vi "Stream to Image Files-example-v2.vi"() -> ()   [LabVIEW 2025]
doc: "The Stream to Image Files example shows how to save images to PNG files in parallel when using a grab acquisition. Images acquired from a camera are stored in a manager and each worker loop removes an image from the manager to save to disk. When the save to disk is complete, the image is added back to the manager so it can be used to copy acquired images into again. It is recommended to use the Stream to Image Files (Optimized Performance) example if your camera settings work with a ring acquisition."
uses:
  VIs_needed/Grab Manager Mode.ctl
  <vilib>/vision/driver/IMAQdx.llb/IMAQdx Buffer Number Mode.ctl
  <vilib>/Utility/High Resolution Relative Seconds.vi
  <vilib>/vision/driver/NI_Vision_Acquisition_Software.lvlib
  <resource>/objmgr/imaqdx.rc
panel:
  out "Images Acquired Per Second":dbl
  in  "Skip Count":u32
  out "Images Behind":i32
  out "Images Saved Per Second":dbl
  in  "Number of Images":u32=30
  out "Destination Folder":path
  out "Write Speed":dbl(graph) caption="Image File Write Speed"
  in  "Camera Name":refnum<k21> caption="IMAQdx Session"
  in  "Stop":bool
  # "Overview: Demonstrates how to stream images to disk in parallel when using a ring acquisition.\nRequirements: Vision Acquisition Software\nInstructions:\n1. Select the Camera Name\n2. Run the VI\n3. Reduce the Number of Workers to see if the streaming of images can keep up with fewer workers.\n4. Increase the Skip Count if Images Behind is greater than 0."
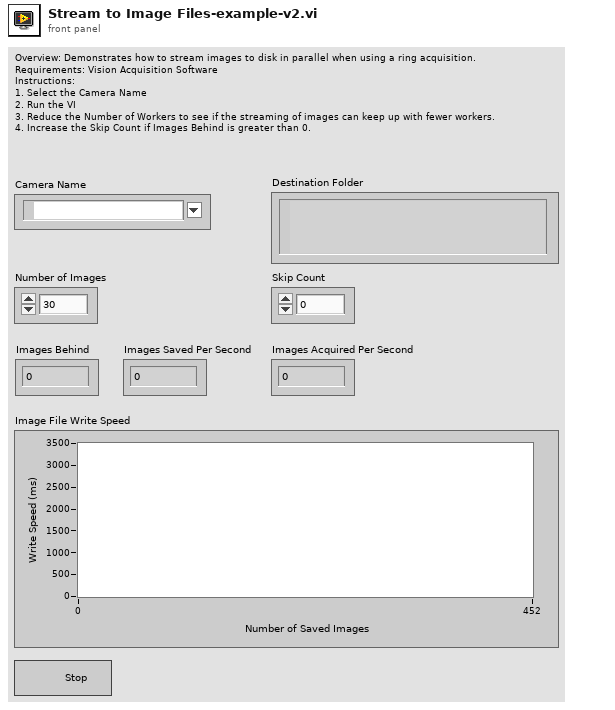
[diagram p1: front panel]
types:
  T1 = cluster{"Number of Processing Images":u32, "Image Border Size":u32}
  T2 = typedef "Grab Manager Mode.ctl" = enum16{"Create Processing Images", "Lock", "Add Acquired Image", "Get Acquired Image", "Unlock", "Dispose Processing Images"}
  T3 = typedef "IMAQdx.ctl" = refnum<k21>
  T4 = typedef "NI_Vision_Acquisition_Software.lvlib/IMAQdx Buffer Number Mode.ctl" = enum32{"Next", "Last", "Buffer Number", "Every", "Last New"}
  T5 = typedef "IMAQ Image.ctl" = refnum<image>
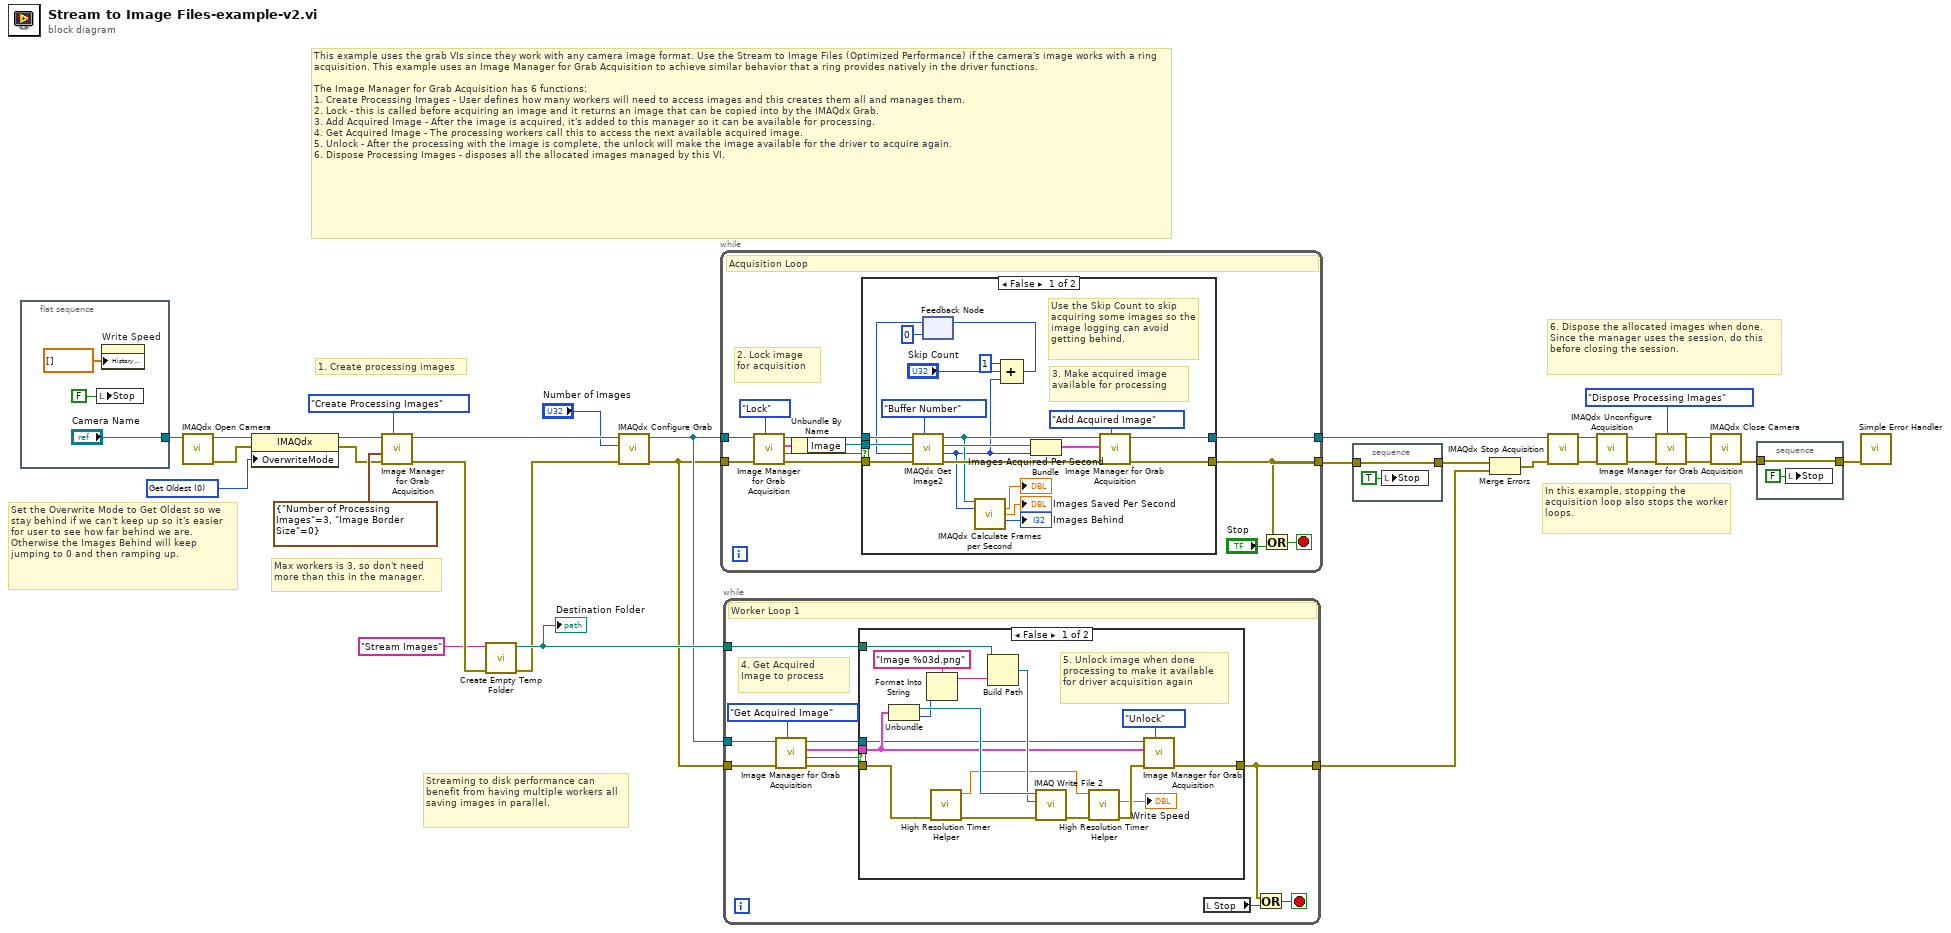
[diagram p0: block diagram]
diagram:
  w19 = u32 0 items=["Get Oldest"=0, "Fail"=2, "Get Newest"=3] ("OverwriteMode")
  # "6. Dispose the allocated images when done. Since the manager uses the session, do this before closing the session."
  # "1. Create processing images"
  # "This example uses the grab VIs since they work with any camera image format. Use the Stream to Image Files (Optimized Performance) if the camera's image works with a ring acquisition. This example uses an Image Manager for Grab Acquisition to achieve similar behavior that a ring provides natively in the driver functions.\n\nThe Image Manager for Grab Acquisition has 6 functions:\n1. Create Processing Images - User defines how many workers will need to access images and this creates them all and manages them.\n2. Lock - this is called before acquiring an image and it returns an image that can be copied into by the IMAQdx Grab.\n3. Add Acquired Image - After the image is acquired, it's added to this manager so it can be available for processing.\n4. Get Acquired Image - The processing workers call this to access the next available acquired image.\n5. Unlock - After the processing with the image is complete, the unlock will make the image available for the driver to acquire again.\n6. Dispose Processing Images - disposes all the allocated images managed by this VI."
  # "Set the Overwrite Mode to Get Oldest so we stay behind if we can't keep up so it's easier for user to see how far behind we are. Otherwise the Images Behind will keep jumping to 0 and then ramping up."
  # "Max workers is 3, so don't need more than this in the manager."
  # "In this example, stopping the acquisition loop also stops the worker loops."
  # "Streaming to disk performance can benefit from having multiple workers all saving images in parallel."
  n1 = flat-sequence {
    tunnel: ["Camera Name"] -> w30
    frame #0 {
      n2 = local write "Stop"(FALSE ("Stop")) -> ()
      n3 = property on="Write Speed" class="WFChart (strict)"("History Data"=dbl[] []) -> ()  [unwired: 2 in, 2 out]
    }
  }
  n4 = call <vilib>:"IMAQdx Open Camera.vi"("Session In"=w30) -> ("error out"=w10:errorcluster, "Session Out"=w20:T3)  [unwired: 2 in, 7 out]
  n5 = property class="IMAQdx"(reference=w20, error in=w10, "OverwriteMode"=w19) -> (reference out=w9:T3, error out=w8:errorcluster)
  n6 = call "Image Manager for Grab Acquisition.vi"("Mode"=Grab_Manager_Mode."Create Processing Images", "error in (no error)"=w8, "Init Settings"=T1 {"Number of Processing Images"=3, "Image Border Size"=0}, "Session In"=w9) -> ("error out"=w7:errorcluster, "Session Out"=w5:T3)  [unwired: 4 in, 2 out]
  n7 = call "Create Empty Temp Folder.vi"("error in (no error)"=w7, "Folder Name"="Stream Images") -> ("error out"=w4:errorcluster, "Empty Temp Folder"=w21:path)  [unwired: 8 in]
  "Destination Folder" <- w21
  n8 = call <vilib>:"IMAQdx Configure Grab.vi"("error in"=w4, "Number of Buffers"="Number of Images", "Session In"=w5) -> ("error out"=w2:errorcluster, "Session Out"=w3:T3)  [unwired: 7 in]
  n9 = while {
    tunnel: w2 -> [w43]
    tunnel: w3 -> [w40]
    tunnel: [w41] -> w26
    tunnel: [w42] -> w25
    stop <- w44 stop-if-true
    # "2. Lock image for acquisition"
    # "Acquisition Loop"
    n10 = call "Image Manager for Grab Acquisition.vi"("Mode"=Grab_Manager_Mode."Lock", "error in (no error)"=w43, "Session In"=w40) -> ("error out"=w36:errorcluster, "No Available Image"=w37:bool, "Image Settings Out"=w35:cluster{"Image":T5, "Buffer Number":u32}, "Session Out"=w38:T3)  [unwired: 5 in]
    n11 = Unbundle By Name(w35) -> ("Image"=w34:T5)
    n12 = case shown="False" w37 {
      tunnel: [w57 w67] -> w41
      tunnel: [w56 w66] -> w42
      tunnel: w38 -> [w65 w67]
      tunnel: w36 -> [w64 w66]
      tunnel: w34 -> [w58 _]
      frame False {
        # "3. Make acquired image available for processing"
        # "Use the Skip Count to skip acquiring some images so the image logging can avoid getting behind."
        n13 = feedback #1(u32 0) -> (w47:u32)
        n14 = call <vilib>:"IMAQdx Get Image2.vi"("Buffer Number Mode (Next)"=IMAQdx_Buffer_Number_Mode."Buffer Number", "error in"=w64, "Buffer Number In"=w47, "Image In"=w58, "Session In"=w65) -> ("error out"=w60:errorcluster, "Buffer Number Out"=w51:u32, "Image Out"=w62:T5, "Session Out"=w55:T3)  [unwired: 3 in]
        n15 = call <vilib>:"IMAQdx Calculate Frames per Second.vi"("Session In"=w55, "Buffer Number"=w51) -> ("Acquired Frames per Second"=→"Images Acquired Per Second":dbl, "Processed Frames per Second"=→"Images Saved Per Second":dbl, "Images Behind"=→"Images Behind":i32)  [unwired: 7 in, 4 out]
        n16 = Compound Arithmetic op=ADD(u32 1 ("value"), "Skip Count", w51) -> (w48:u32)
        n17 = feedback-in #1(w48) -> ()
        n18 = Bundle("Image Out"=w62, "Buffer Number Out"=w51) -> (w61:cluster{"Image Out":T5, "Buffer Number Out":u32})  [unwired: 1 in]
        n19 = call "Image Manager for Grab Acquisition.vi"("Mode"=Grab_Manager_Mode."Add Acquired Image", "error in (no error)"=w60, "Image Settings In"=w61, "Session In"=w55) -> ("error out"=w56:errorcluster, "Session Out"=w57:T3)  [unwired: 4 in, 2 out]
      }
      frame True {
        # "The Lock function already has a delay inside when no images are available to prevent loop from going too fast and starving the worker threads from getting processing time."
        # "Write to disk operation is taking longer so images aren't added back to manager. Wait until there is an available image"
      }
    }
    n20 = Or(x=w42, y="Stop") -> (x .or. y?=w44:bool)
  }
  n21 = while {
    tunnel: w2 -> [w74]
    tunnel: w21 -> [w76]
    tunnel: [w75] -> w22
    tunnel: w3 -> [w69]
    stop <- w78 stop-if-true
    # "4. Get Acquired Image to process"
    # "Worker Loop 1"
    n22 = call "Image Manager for Grab Acquisition.vi"("Mode"=Grab_Manager_Mode."Get Acquired Image", "error in (no error)"=w74, "Session In"=w69) -> ("error out"=w70:errorcluster, "No Available Image"=w72:bool, "Image Settings Out"=w71:cluster{"Image":T5, "Buffer Number":u32}, "Session Out"=w68:T3)  [unwired: 5 in]
    n23 = case shown="False" w72 {
      tunnel: w70 -> [w84 w95]
      tunnel: w71 -> [w86 _]
      tunnel: [w88 w95] -> w75
      tunnel: w76 -> [w93 _]
      tunnel: w68 -> [w85 _]
      frame False {
        # "5. Unlock image when done processing to make it available for driver acquisition again"
        n24 = Unbundle(w86) -> ("Image"=w94:T5, "Buffer Number"=w90:u32)
        n25 = Format Into String(format string="Image %03d.png", w90) -> (resulting string=w92:string)  [unwired: 2 in, 1 out]
        n26 = call "High Resolution Timer Helper.vi"("error in (no error)"=w84) -> ("error out"=w83:errorcluster, "Current Time"=w80:dbl)  [unwired: 8 in, 1 out]
        n27 = Build Path(base path=w93, name or relative path=w92) -> (appended path=w89:path)
        n28 = call-poly "IMAQ Write File 2"("error in (no error)"=w83, "File Path"=w89, "Image"=w94) -> ("error out"=w82:errorcluster)  [unwired: 7 in, 1 out]
        n29 = call "High Resolution Timer Helper.vi"("error in (no error)"=w82, "Previous Time"=w80) -> ("error out"=w81:errorcluster, "Time Difference (ms)"=→"Write Speed":dbl)  [unwired: 7 in, 1 out]
        n30 = call "Image Manager for Grab Acquisition.vi"("Mode"=Grab_Manager_Mode."Unlock", "error in (no error)"=w81, "Image Settings In"=w86, "Session In"=w85) -> ("error out"=w88:errorcluster)  [unwired: 4 in, 3 out]
      }
      frame True {
        # "No acquired images to process"
      }
    }
    n31 = local read "Stop"() -> (w77:bool)
    n32 = Or(x=w75, y=w77) -> (x .or. y?=w78:bool)
  }
  n33 = stacked-sequence {
    tunnel: [w96] -> w24
    tunnel: w25 -> [w96]
    frame #0 {
      n34 = local write "Stop"(TRUE ("Stop")) -> ()
    }
  }
  n35 = Merge Errors(w24, w22) -> (w27:errorcluster)
  n36 = call <vilib>:"IMAQdx Stop Acquisition.vi"("error in"=w27, "Session In"=w26) -> ("error out"=w28:errorcluster, "Session Out"=w29:T3)  [unwired: 8 out]
  n37 = call <vilib>:"IMAQdx Unconfigure Acquisition.vi"("error in"=w28, "Session In"=w29) -> ("error out"=w17:errorcluster, "Session Out"=w18:T3)  [unwired: 8 out]
  n38 = call "Image Manager for Grab Acquisition.vi"("Mode"=Grab_Manager_Mode."Dispose Processing Images", "error in (no error)"=w17, "Session In"=w18) -> ("error out"=w14:errorcluster, "Session Out"=w15:T3)  [unwired: 5 in, 2 out]
  n39 = call <vilib>:"IMAQdx Close Camera.vi"("error in"=w14, "Session In"=w15) -> ("error out"=w13:errorcluster)  [unwired: 9 out]
  n40 = stacked-sequence {
    tunnel: [w98] -> w23
    tunnel: w13 -> [w98]
    frame #0 {
      n41 = local write "Stop"(FALSE ("Stop")) -> ()
    }
  }
  n42 = call <vilib>:"Simple Error Handler.vi"("error in (no error)"=w23) -> ()  [unwired: 4 in, 5 out]
